vi "Alerte Ecart temperature.vi"() -> ()   [LabVIEW 2022 SP3]
uses:
  Enum/Enum 2.ctl
  Variables globales/Variables glob EUROTHERM.vi
  Variables globales/Variable glob Th.vi
  Variables globales/Variable glob Pt.vi
  Variables globales/Variable glob alertes ecart temperatures.vi
panel:
  out "Nb pages":u8
  in  "ajouter":bool
  in  "Groupes":T1(array[cluster])=[{"Capteurs"=[5], "Ecart"=5.0, "Alerte"=FALSE, ">?"=TRUE, "N°"=0}] caption="Groupes alertes ecarts temperatures" {"Ecart" min=0.0 format="%.2g"}
  in  "OK":bool
  in  "Annuler":bool
  # "PARAMeTRES POUR ALERTE ecart TEMPeRATURE PAR ENVOI D'UN MAIL"
  # "Ce logiciel et les informations qu'il contient, sont la propriété de l’IAS et ne peuvent être diffusés sans l’autorisation de la Station d’étalonnage"
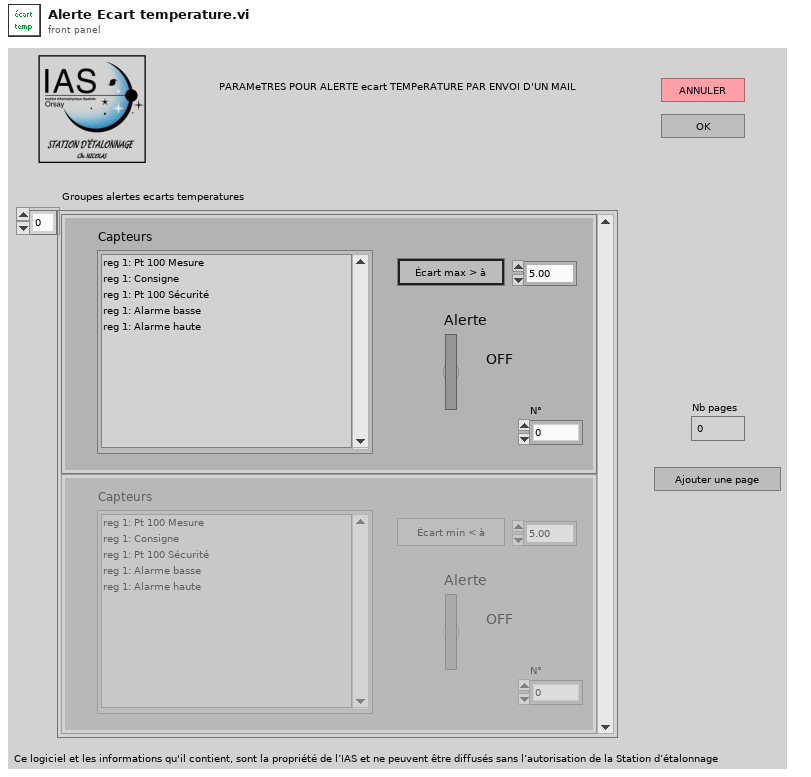
[diagram p1: front panel]
types:
  T1 = cluster{"Capteurs":i32[], "Ecart":dbl, "Alerte":bool, ">?":bool, "N°":u16}[]
  T2 = typedef "Enum 2.ctl" = enum16{"init noms", "initialisation", "choix", "GO"}
  T3 = cluster{"Noms voies select acqui 1COM":string[]}[]
  T4 = cluster{"Nom tache Pt":refnum<k21>, "Noms des Pt":string[], "Nb Pt":i16, "Selection Pt":bool[], "Nom Pt selectionnees":string[]}[]
  T5 = cluster{"Nom tache Th":refnum<k21>, "Noms des Th":string[], "Nb Th":i16, "Selection Th":bool[], "Nom Th selectionnes":string[]}[]
  T6 = cluster{"Indices a controler":i16[], "Defaut":bool, "ecart temp":dbl, "Alerte":bool, ">?":bool, "N°":u16}[]
  T7 = cluster{"Capteurs":i32[], "Ecart":dbl, "Alerte":bool, ">?":bool, "N°":u16}
  T8 = cluster{"Indices a controler":i16[], "Defaut":bool, "ecart temp":dbl, "Alerte":bool, ">?":bool, "N°":u16}
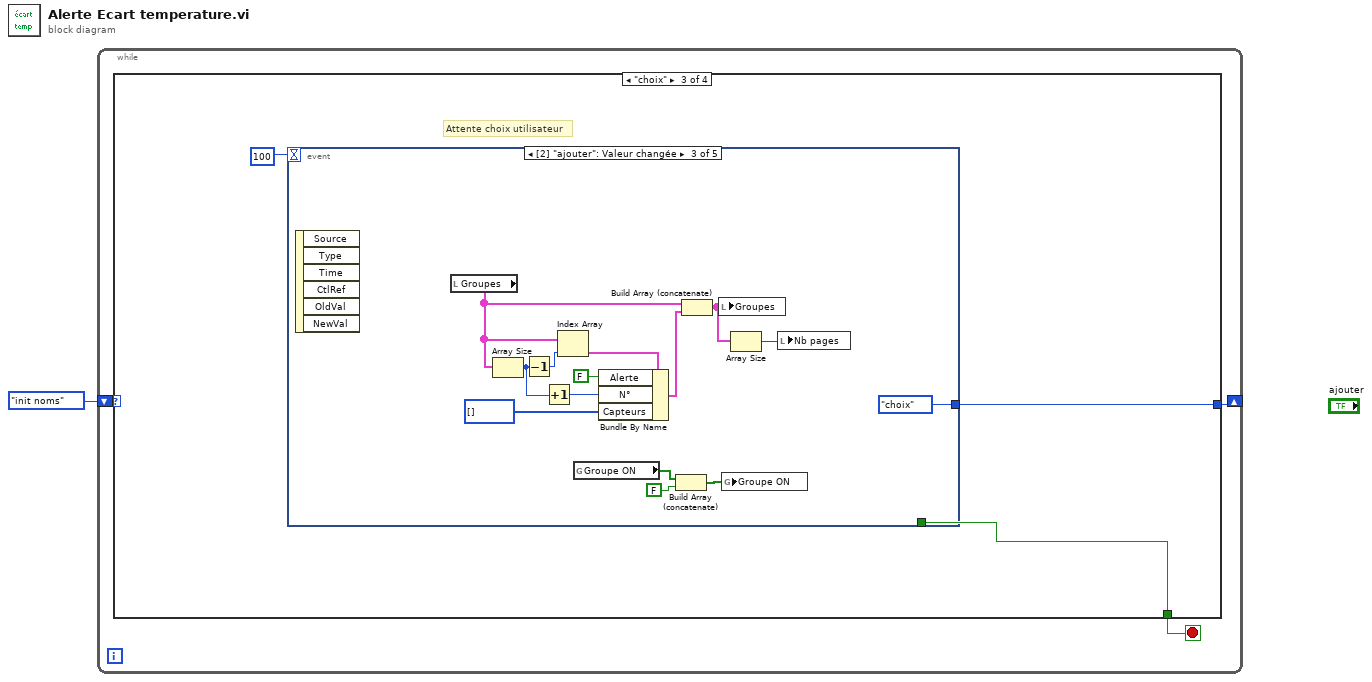
[diagram p0: block diagram]
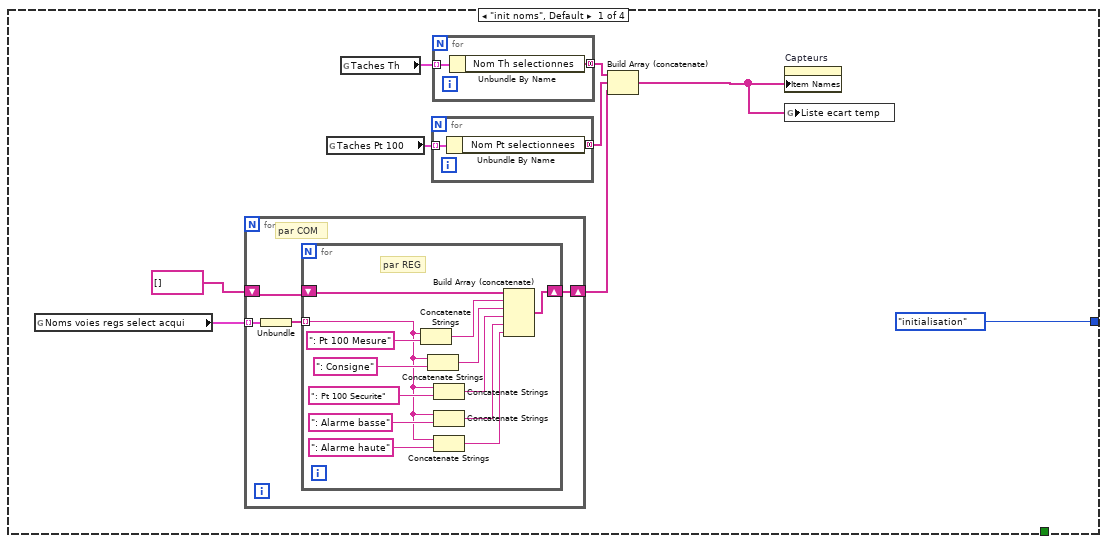
[diagram p2: hidden frame]
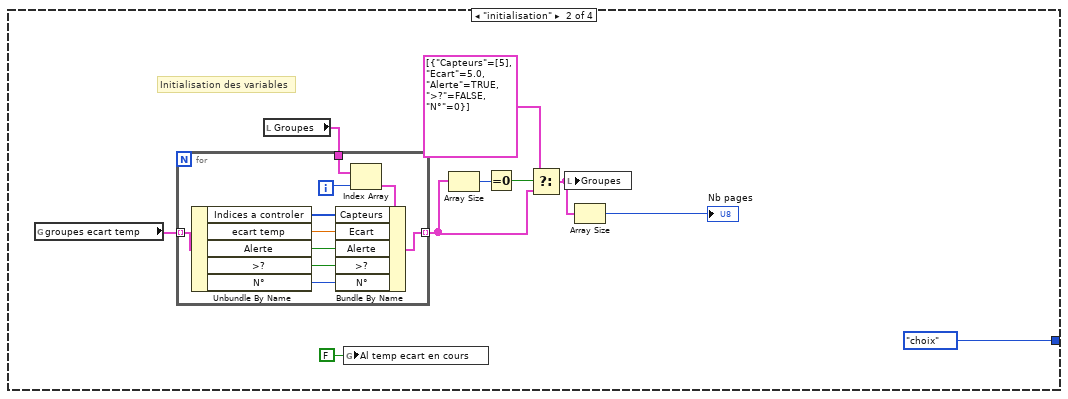
[diagram p3: hidden frame]
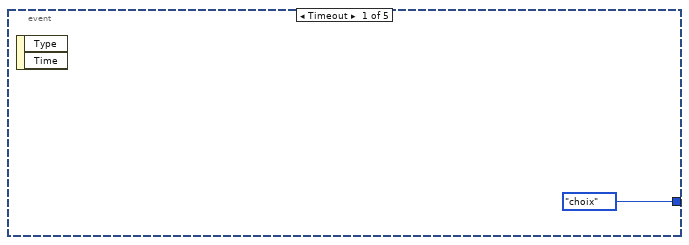
[diagram p4: hidden frame]
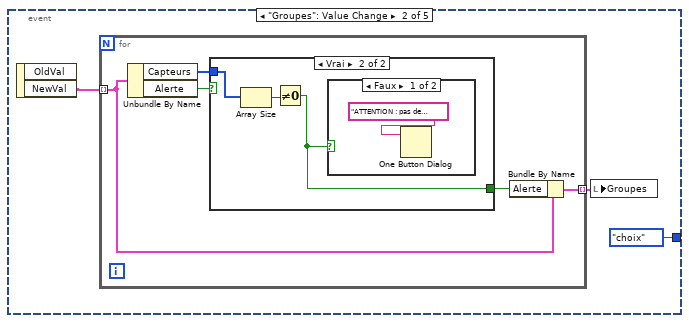
[diagram p5: hidden frame]
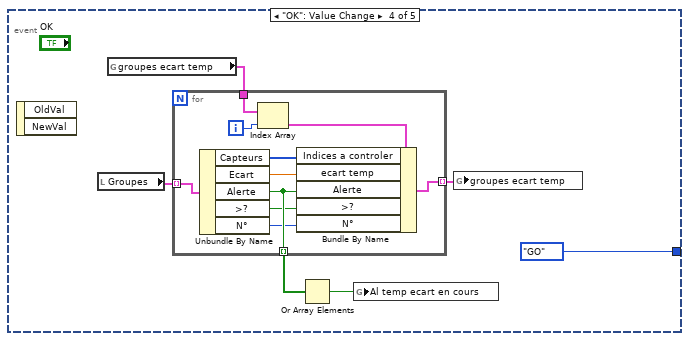
[diagram p8: hidden frame]
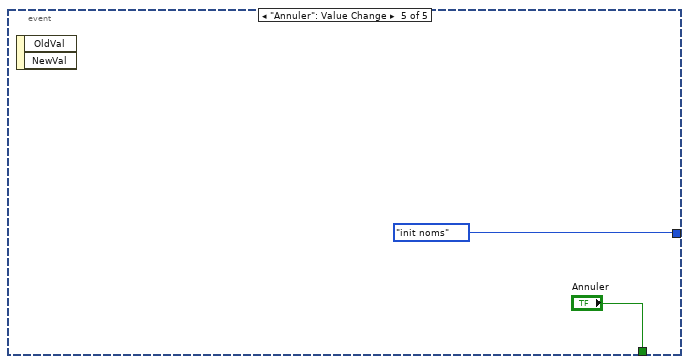
[diagram p9: hidden frame]
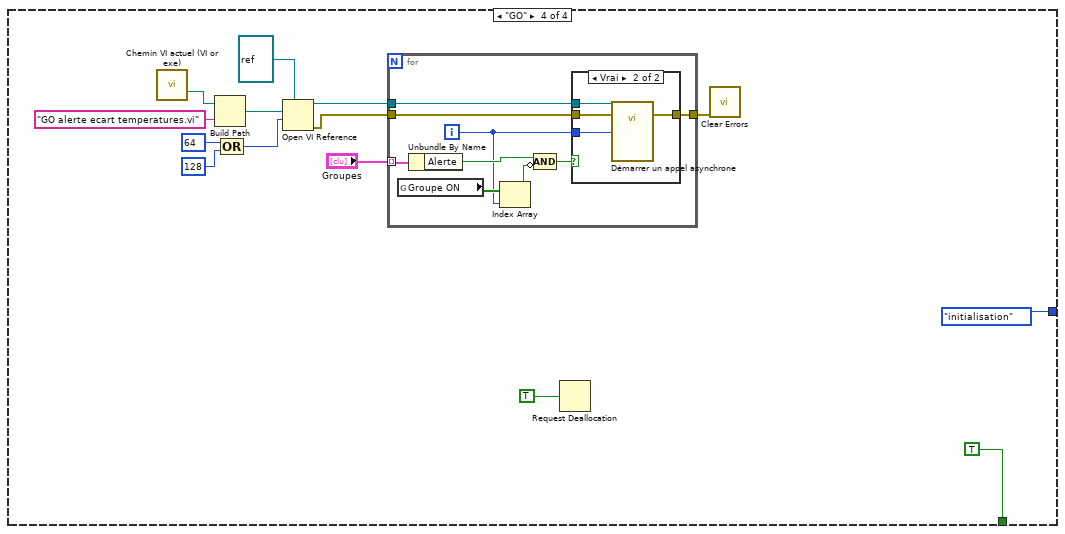
[diagram p10: hidden frame]
diagram:
  n1 = while {
    shift-right: [w3] -> _
    shift-left: Enum_2."init noms" ("Énum") -> [w4]
    stop <- w2 stop-if-true
    n2 = case shown="\"choix\"" w4 {
      tunnel: [Enum_2."initialisation" ("Énum") Enum_2."choix" ("Énum") w55 Enum_2."initialisation" ("Énum")] -> w3
      tunnel: [_ _ w56 TRUE] -> w2
      frame "init noms", Default {
        n3 = global read "Variables glob EUROTHERM.vi" "Noms voies regs select acqui"() -> (w11:T3)
        n4 = for {
          tunnel: w11 -> [w18] mode=indexing
          shift-right: [w21] -> w6
          shift-left: string[] [] -> [w19]
          # "par COM"
          n5 = Unbundle(w18) -> ("Noms voies select acqui 1COM"=w20:string[])
          n6 = for {
            tunnel: w20 -> [w24] mode=indexing
            shift-right: [w30] -> w21
            shift-left: w19 -> [w34]
            # "par REG"
            n7 = Concatenate Strings(w24, ": Pt 100 Mesure") -> (w31:string)
            n8 = Concatenate Strings(w24, ": Consigne") -> (w28:string)
            n9 = Concatenate Strings(w24, ": Pt 100 Securite") -> (w26:string)
            n10 = Concatenate Strings(w24, ": Alarme basse") -> (w23:string)
            n11 = Concatenate Strings(w24, ": Alarme haute") -> (w22:string)
            n12 = Build Array (concatenate)(w34, w31, w28, w26, w23, w22) -> (w30:string[])
          }
        }
        n13 = global read "Variable glob Pt.vi" "Taches Pt 100"() -> (w10:T4)
        n14 = global read "Variable glob Th.vi" "Taches Th"() -> (w7:T5)
        n15 = for {
          tunnel: w10 -> [w17] mode=indexing
          tunnel: [w16] -> w9 mode=concatenating
          n16 = Unbundle By Name(w17) -> ("Nom Pt selectionnees"=w16:string[])
        }
        n17 = for {
          tunnel: w7 -> [w15] mode=indexing
          tunnel: [w14] -> w8 mode=concatenating
          n18 = Unbundle By Name(w15) -> ("Nom Th selectionnes"=w14:string[])
        }
        n19 = Build Array (concatenate)(w8, w9, w6) -> (w5:string[])
        n20 = property on="Capteurs" class="LstDér (strict)"("Item Names"=w5) -> ()  [unwired: 2 in, 2 out]
        n21 = global write "Variable glob alertes ecart temperatures.vi" "Liste ecart temp"(w5) -> ()
      }
      frame "initialisation" {
        # "Initialisation des variables"
        n22 = global read "Variable glob alertes ecart temperatures.vi" "groupes ecart temp"() -> (w42:T6)
        n23 = local read "Groupes"() -> (w43:T1)
        n24 = for {
          tunnel: w42 -> [w54] mode=indexing
          tunnel: w43 -> [w53]
          tunnel: [w48] -> w39 mode=indexing
          i -> [w47]
          n25 = Unbundle By Name(w54) -> ("Indices a controler"=w49:i16[], "ecart temp"=w51:dbl, "Alerte"=w50:bool, ">?"=w46:bool, "N°"=w45:u16)
          n26 = Index Array(array=w53, index=w47) -> (element=w52:T7)
          n27 = Bundle By Name(cluster=w52, "Capteurs"=w49, "Ecart"=w51, "Alerte"=w50, ">?"=w46, "N°"=w45) -> (w48:T7)
        }
        n28 = global write "Variable glob alertes ecart temperatures.vi" "Al temp ecart en cours"(FALSE ("Al temp ecart en cours")) -> ()
        n29 = Array Size(array=w39) -> (size(s)=w41:i32)
        n30 = Equal To 0?(x=w41) -> (x = 0?=w40:bool)
        n31 = Select(t=T1 [{"Capteurs"=[5], "Ecart"=5.0, "Alerte"=TRUE, ">?"=FALSE, "N°"=0}] ("cas vrai"), s=w40, f=w39) -> (s? t:f=w38:T1)
        n32 = local write "Groupes"(w38) -> ()
        n33 = Array Size(array=w38) -> (size(s)=→"Nb pages":i32)
      }
      frame "choix" {
        # "Attente choix utilisateur"
        n34 = event shown="[2] \"ajouter\": Valeur changée" {
          selector: _ -> [_ _ _ _ _]
          dyn-events: _ -> [_ _ _ _ _]
          timeout: 100 -> [_ _ _ _ _]
          tunnel: [_ _ _ _ "Annuler"] -> w56
          tunnel: [Enum_2."choix" ("Énum") Enum_2."choix" ("Énum") Enum_2."choix" ("Énum") Enum_2."GO" ("Énum") Enum_2."init noms" ("Énum")] -> w55
          event Timeout {
            n35 = event-data() -> ()  [unwired: 1 in, 2 out]
          }
          event "Groupes": Value Change {
            n36 = event-data() -> ("NewVal"=w60:T1)  [unwired: 1 in, 1 out]
            n37 = for {
              tunnel: w60 -> [w65] mode=indexing
              tunnel: [w62] -> w59 mode=indexing
              n38 = Unbundle By Name(w65) -> ("Capteurs"=w64:i32[], "Alerte"=w66:bool)
              n39 = case shown="Vrai" w66 {
                selector: w66 -> [w67 _]
                tunnel: w64 -> [_ w70]
                tunnel: [w67 w68] -> w63
                frame False {
                }
                frame True {
                  n40 = Array Size(array=w70) -> (size(s)=w69:i32)
                  n41 = Not Equal To 0?(x=w69) -> (x != 0?=w68:bool)
                  n42 = case shown="Faux" w68 {
                    frame False {
                      n43 = One Button Dialog(message="ATTENTION : pas de capteur choisi dans la liste") -> ()  [unwired: 1 in, 1 out]
                    }
                    frame True {
                    }
                  }
                }
              }
              n44 = Bundle By Name(cluster=w65, "Alerte"=w63) -> (w62:T7)
            }
            n45 = local write "Groupes"(w59) -> ()
          }
          event "ajouter": Value Change {
            n46 = event-data() -> ()  [unwired: 1 in, 6 out]
            n47 = local read "Groupes"() -> (w82:T1)
            n48 = Array Size(array=w82) -> (size(s)=w74:i32)
            n49 = Decrement(x=w74) -> (x-1=w81:i32)
            n50 = Increment(x=w74) -> (x+1=w73:i32)
            n51 = Index Array(array=w82, index=w81) -> (element=w83:T7)
            n52 = global read "Variable glob alertes ecart temperatures.vi" "Groupe ON"() -> (w77:bool[])
            n53 = Bundle By Name(cluster=w83, "Alerte"=FALSE, "N°"=w73, "Capteurs"=i32[] []) -> (w85:T7)
            n54 = Build Array (concatenate)(w77, FALSE) -> (w75:bool[])
            n55 = Build Array (concatenate)(w82, w85) -> (w79:T1)
            n56 = local write "Groupes"(w79) -> ()
            n57 = global write "Variable glob alertes ecart temperatures.vi" "Groupe ON"(w75) -> ()
            n58 = Array Size(array=w79) -> (size(s)=w78:i32)
            n59 = local write "Nb pages"(w78) -> ()
          }
          event "OK": Value Change {
            n60 = event-data() -> ()  [unwired: 1 in, 2 out]
            n61 = local read "Groupes"() -> (w88:T1)
            n62 = global read "Variable glob alertes ecart temperatures.vi" "groupes ecart temp"() -> (w90:T6)
            n63 = for {
              tunnel: w88 -> [w101] mode=indexing
              tunnel: w90 -> [w100]
              tunnel: [w95] -> w89 mode=indexing
              tunnel: [w94] -> w86 mode=indexing
              i -> [w99]
              n64 = Unbundle By Name(w101) -> ("Capteurs"=w97:i32[], "Ecart"=w96:dbl, "Alerte"=w94:bool, ">?"=w93:bool, "N°"=w92:u16)
              n65 = Index Array(array=w100, index=w99) -> (element=w98:T8)
              n66 = Bundle By Name(cluster=w98, "Indices a controler"=w97, "ecart temp"=w96, "Alerte"=w94, ">?"=w93, "N°"=w92) -> (w95:T8)
            }
            n67 = Or Array Elements(Boolean array=w86) -> (logical OR=w87:bool)
            n68 = global write "Variable glob alertes ecart temperatures.vi" "Al temp ecart en cours"(w87) -> ()
            n69 = global write "Variable glob alertes ecart temperatures.vi" "groupes ecart temp"(w89) -> ()
          }
          event "Annuler": Value Change {
            n70 = event-data() -> ()  [unwired: 1 in, 2 out]
          }
        }
      }
      frame "GO" {
        n71 = call "Chemin VI actuel (VI or exe).vi"() -> ("VI or executable installation directory"=w109:path)  [unwired: 14 in, 1 out]
        n72 = Build Path(base path=w109, name or relative path="GO alerte ecart temperatures.vi" ("nom ou chemin relatif")) -> (appended path=w114:path)
        n73 = Compound Arithmetic op=OR(64 ("options"), 128 ("options")) -> (w110:i32)
        n74 = Open VI Reference(type specifier VI Refnum (for type only)=refnum<vi> refnum ("spécificateur de type du refnum de VI (pour type seulement)"), vi path=w114, options=w110) -> (vi reference=w108:refnum<vi>, error out=w107:errorcluster)  [unwired: 3 in]
        n75 = for {
          tunnel: w108 -> [w124]
          tunnel: w107 -> [w126]
          tunnel: [w125] -> w105
          tunnel: "Groupes" -> [w123] mode=indexing
          i -> [w119]
          n76 = global read "Variable glob alertes ecart temperatures.vi" "Groupe ON"() -> (w120:bool[])
          n77 = Unbundle By Name(w123) -> ("Alerte"=w122:bool)
          n78 = Index Array(array=w120, index=w119) -> (element=w118:bool)
          n79 = Compound Arithmetic op=AND ("Opérateur arithmétique")(w122, invert w118) -> (w121:bool)
          n80 = case shown="Vrai" w121 {
            tunnel: w126 -> [w127 w131]
            tunnel: [w127 w130] -> w125
            tunnel: w124 -> [_ w128]
            tunnel: w119 -> [_ w129]
            frame False {
            }
            frame True {
              n81 = call-by-ref "Démarrer un appel asynchrone"(reference=w128, error in=w131, "Numéro"=w129) -> (error out=w130:errorcluster)  [unwired: 2 in, 2 out]
            }
          }
        }
        n82 = Request Deallocation(TRUE ("flag")) -> ()
        n83 = call <vilib>:"Clear Errors.vi"("error in (no error)"=w105) -> ()  [unwired: 5 in, 2 out]
      }
    }
  }
